vi "libssh2_channel_open_ex.vi"(5 "packet_size (32 KiB)":u32=32768, 7 "window_size (2 MiB)":u32=2097152, 8 "error in (no error)":errorcluster, 9 "message":string, 10 "channel_type":string="session", 11 "session":T1) -> (0 "error out":errorcluster, 3 "channel":T2)   [LabVIEW 2017, in "libssh2.lvlib"]
doc: "Open a channel."
uses:
  libssh2.lvlib
  Channel Refnum.ctl
  Session Refnum.ctl
  Not A Session.vi
  <vilib>/Utility/error.llb/Error Cluster From Error Code.vi
  Global Settings.vi
  Read Session Refnum.vi
  <vilib>/Utility/semaphor.llb/Acquire Semaphore.vi
  <vilib>/Utility/semaphor.llb/Release Semaphore.vi
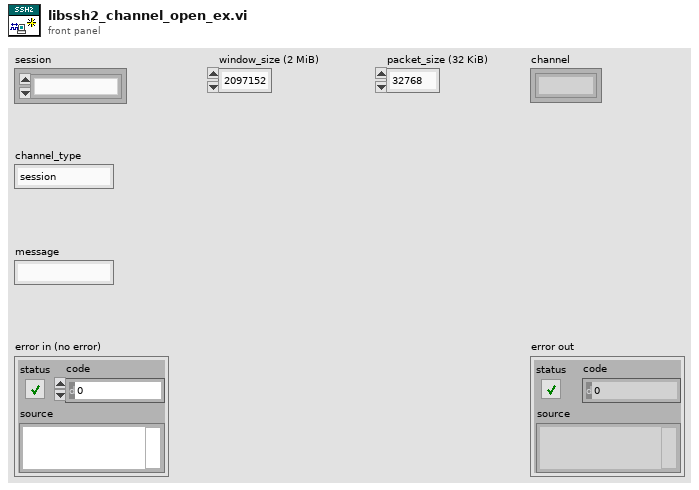
[diagram p1: front panel]
types:
  T1 = typedef "libssh2.lvlib/Session Refnum.ctl" = refnum<k1>
  T2 = typedef "libssh2.lvlib/Channel Refnum.ctl" = refnum<k1>
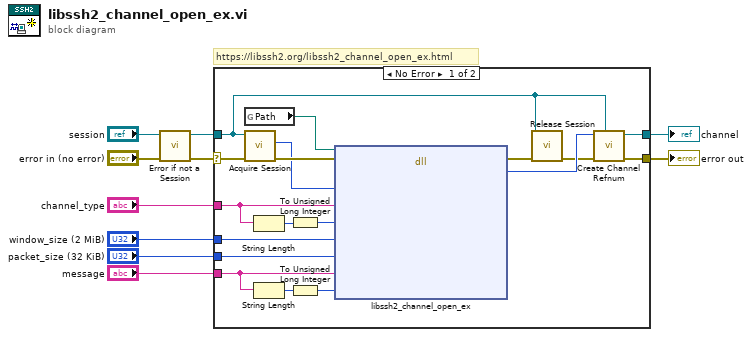
[diagram p0: block diagram]
diagram:
  # "https://libssh2.org/libssh2_channel_open_ex.html"
  n1 = call "Error if not a Session.vi"("error in (no error)"="error in (no error)", "session"="session") -> ("error out"=w3:errorcluster, "session out"=w1:T1)  [unwired: 8 in]
  n2 = case shown="No Error" w3 {
    selector: w3 -> [w14 w29]
    tunnel: "window_size (2 MiB)" -> [w27 _]
    tunnel: "packet_size (32 KiB)" -> [w26 _]
    tunnel: "message" -> [w24 _]
    tunnel: "channel_type" -> [w22 _]
    tunnel: w1 -> [w11 _]
    tunnel: [w17 w29] -> w6
    tunnel: [w15 _] -> w5
    frame No Error {
      n3 = global read "Global Settings.vi" "Path"() -> (w13:path)
      n4 = call "Acquire Session.vi"("error in (no error)"=w14, "session"=w11) -> ("error out"=w19:errorcluster, "LIBSSH2_SESSION*"=w18:u64)  [unwired: 7 in, 1 out]
      n5 = String Length(string=w22) -> (length=w20:i32)
      n6 = String Length(string=w24) -> (length=w21:i32)
      n7 = To Unsigned Long Integer(number=w20) -> (unsigned 32bit integer=w28:u32)
      n8 = To Unsigned Long Integer(number=w21) -> (unsigned 32bit integer=w23:u32)
      n9 = dll-call lib="?" fn="libssh2_channel_open_ex"(path in=w13, error in=w19, "session"=w18, "channel_type"=w22, "channel_type_len"=w28, "window_size"=w27, "packet_size"=w26, "message"=w24, "message_len"=w23) -> (error out=w25:errorcluster, "return value"=w16:u64)  [unwired: 8 in, 1 out]
      n10 = call "Release Session.vi"("error in (no error)"=w25, "session"=w11) -> ("error out"=w12:errorcluster)  [unwired: 9 in]
      n11 = call "Create Channel Refnum.vi"("session"=w11, "error in (no error)"=w12, "LIBSSH2_CHANNEL*"=w16) -> ("error out"=w17:errorcluster, "channel"=w15:T2)  [unwired: 7 in]
    }
    frame Error {
    }
  }
  "channel" <- w5
  "error out" <- w6
